vi "Measurement Logic.vi"() -> ()   [LabVIEW 2021, in "SourceMeasureDCVoltage.lvlib"]
uses:
  SourceMeasureDCVoltage.lvlib
  FAL/Functions/Measure_Voltage/Measure_Voltage.lvclass
  FAL/Functions/Source_Voltage/Source_Voltage.lvclass
  FAL/Instruments/Abstract_Instrument/Abstract_Instrument.lvclass
  Measurement Results.ctl
  FAL/Instruments/Abstract_Instrument/controls/Initialize_Info.ctl
  FAL/Instruments/Abstract_Instrument/Utility/Initialize N Pins.vi
  FAL/Functions/Measure_Voltage/Utility/Get 1 Object.vi
  FAL/Functions/Source_Voltage/Utility/Get 1 Object.vi
  <vilib>/Plug-In SDKs/Clients/Session Management V1/Session Reservation/Initialize and Close Session Behavior.ctl
  <vilib>/Plug-In SDKs/Clients/Session Management V1/Session Reservation/Session Reservation.lvclass
  3a97cad3-1174-4d4c-995c-4f8f4017f4b7.vi
  Measurement Configuration.ctl
  <vilib>/Plug-In SDKs/Measurements/Measure Call Context/Measure Call Context.lvclass
panel:
  out "measure call context out":refnum<class "Measure Call Context.lvclass">
  in  "measure call context in":refnum<class "Measure Call Context.lvclass">
  in  "measurement configuration":T1={"source_pin"="", "Voltage Level"=0.0, "Voltage Level Range"=0.0, "Current Limit"=0.0, "Current Limit Range"=0.0, "Source Delay (Sec)"=0.0, "measure_pin"="", "Resolution in Digits"=enum."5 1/2"}
  out "measurement results":T2 {"Measurement" format="%.6p"}
  out "error out":errorcluster
  in  "error in":errorcluster
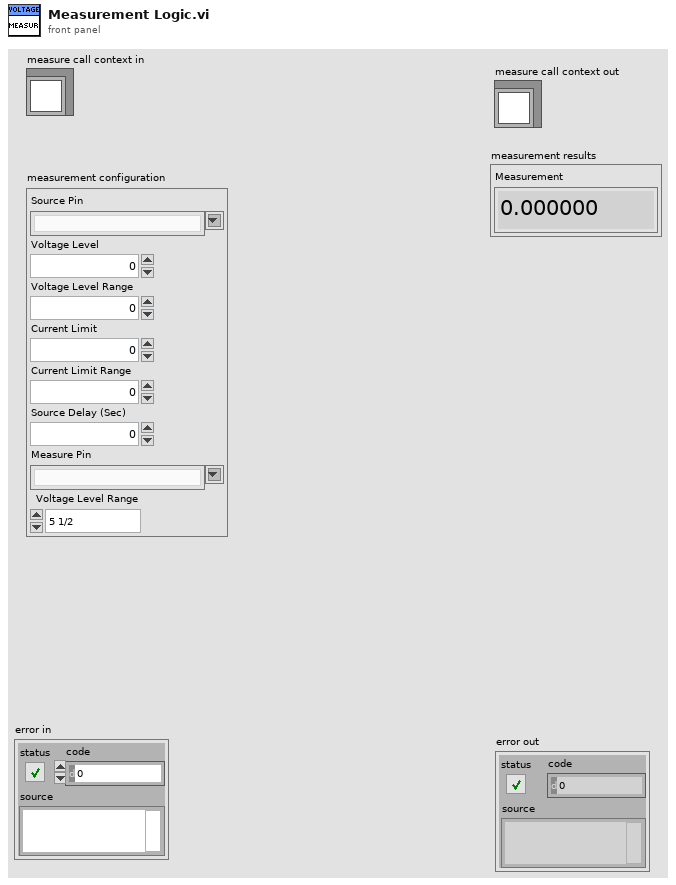
[diagram p1: front panel]
types:
  T1 = typedef "SourceMeasureDCVoltage.lvlib/Measurement Configuration.ctl" = cluster{"source_pin":string, "Voltage Level":dbl, "Voltage Level Range":dbl, "Current Limit":dbl, "Current Limit Range":dbl, "Source Delay (Sec)":dbl, "measure_pin":string, "Resolution in Digits":enum32{"3 1/2", "4 1/2", "5 1/2", "6 1/2", "7 1/2"}}
  T2 = typedef "SourceMeasureDCVoltage.lvlib/Measurement Results.ctl" = cluster{"Measurement":dbl}
  T3 = typedef "NI Session Management V1 Client.lvlib/Session Reservation.lvclass/Initialize and Close Session Behavior.ctl" = enum16{"Auto", "Initialize and Close", "Attach and Detach", "Initialize and Detach", "Attach and Close"}
  T4 = typedef "Abstract_Instrument.lvclass/Initialize_Info.ctl" = cluster{"initialize and close session behavior":T3, "reset":bool, "optional string":string}
  T5 = enum32{"3 1/2", "4 1/2", "5 1/2", "6 1/2", "7 1/2"}
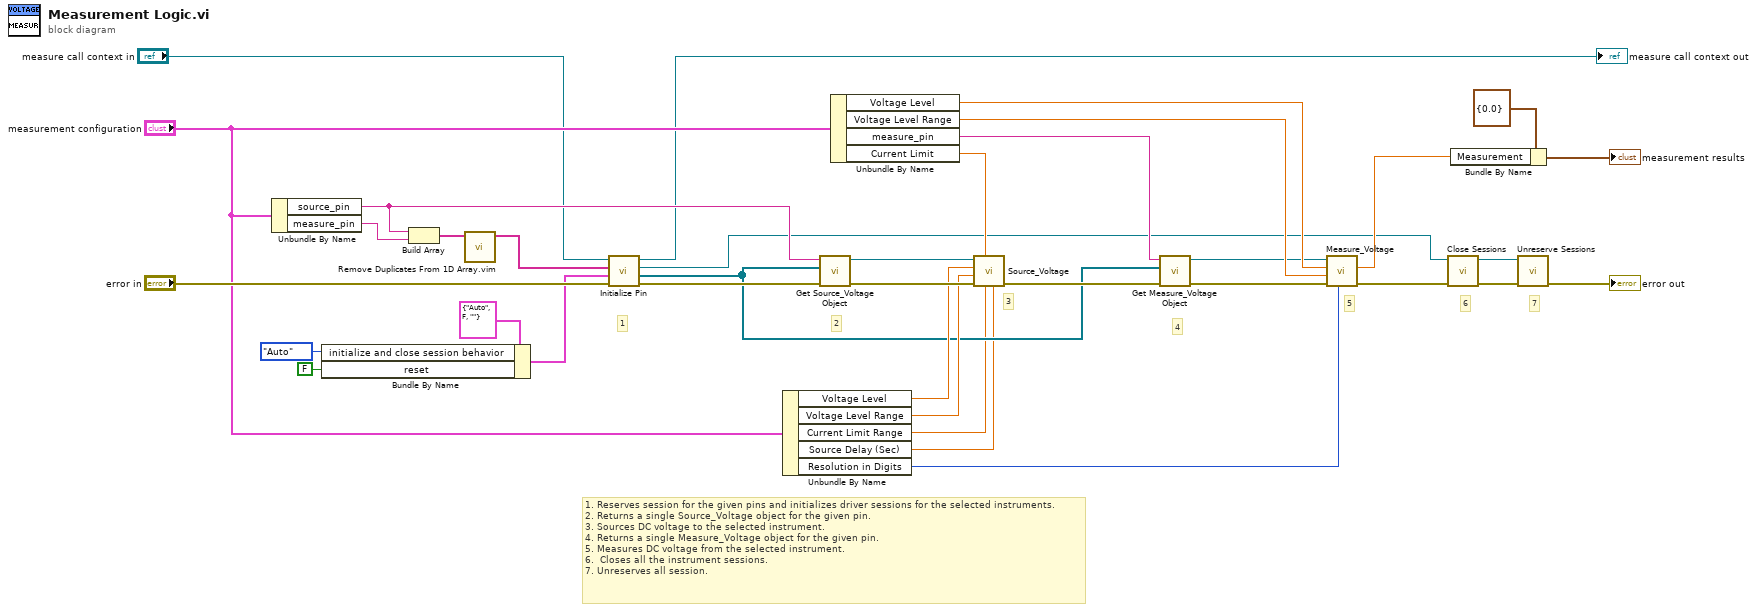
[diagram p0: block diagram]
diagram:
  # "1. Reserves session for the given pins and initializes driver sessions for the selected instruments.\n2. Returns a single Source_Voltage object for the given pin.\n3. Sources DC voltage to the selected instrument.\n4. Returns a single Measure_Voltage object for the given pin.\n5. Measures DC voltage from the selected instrument.\n6.  Closes all the instrument sessions.\n7. Unreserves all session."
  # "7"
  # "6"
  # "5"
  # "4"
  # "3"
  # "2"
  # "1"
  n1 = Unbundle By Name("measurement configuration") -> ("source_pin"=w24:string, "measure_pin"=w27:string)
  n2 = Bundle By Name(cluster=T4 {"initialize and close session behavior"=enum."Auto", "reset"=FALSE, "optional string"=""} ("Initialize_Info"), "initialize and close session behavior"=Initialize_and_Close_Session_Behavior."Auto", "reset"=FALSE) -> (w14:T4)
  n3 = Build Array(w24, w27) -> (w25:string[])
  n4 = call "Remove Duplicates From 1D Array.vim"("array"=w25) -> ("array with duplicates removed"=w6:string[])  [unwired: 10 in]
  n5 = call-poly "Initialize Pin.vi"("error in"="error in", "Initialize_Info"=w14, "pin or relay names"=w6, "measure call context in"="measure call context in") -> ("error out"=w26:errorcluster, "instrument object"=w21:refnum<class "Abstract_Instrument.lvclass">[], "session reservation out"=w2:refnum<class "Session Reservation.lvclass">, "measure call context out"=→"measure call context out":refnum<class "Measure Call Context.lvclass">)  [unwired: 4 in]
  n6 = Unbundle By Name("measurement configuration") -> ("Voltage Level"=w29:dbl, "Voltage Level Range"=w28:dbl, "Current Limit Range"=w11:dbl, "Source Delay (Sec)"=w10:dbl, "Resolution in Digits"=w5:T5)
  n7 = call-poly "Get Source_Voltage Object.vi"("error in"=w26, "instrument object"=w21, "pin_name"=w24) -> ("error out"=w31:errorcluster, "function object"=w23:refnum<class "Source_Voltage.lvclass">)  [unwired: 7 in]
  n8 = Unbundle By Name("measurement configuration") -> ("Voltage Level"=w4:dbl, "Voltage Level Range"=w3:dbl, "measure_pin"=w22:string, "Current Limit"=w12:dbl)
  n9 = call-dynamic "Source_Voltage.vi"("Source Delay (Sec)"=w10, "Current Limit Range"=w11, "Current Limit"=w12, "error in (no error)"=w31, "Voltage Level Range"=w28, "Voltage Level"=w29, "Source_Voltage in"=w23) -> ("error out"=w30:errorcluster)  [unwired: 3 in, 1 out]
  n10 = call-poly "Get Measure_Voltage Object.vi"("error in"=w30, "instrument object"=w21, "pin_name"=w22) -> ("error out"=w32:errorcluster, "function object"=w1:refnum<class "Measure_Voltage.lvclass">)  [unwired: 7 in]
  n11 = call-dynamic "Measure_Voltage.vi"("Resolution in Digits"=w5, "error in (no error)"=w32, "Range"=w3, "Level"=w4, "Measure_Voltage in"=w1) -> ("error out"=w34:errorcluster, "DC_Voltage"=w33:dbl)  [unwired: 3 in, 2 out]
  n12 = call <vilib>:"Close Sessions.vi"("error in"=w34, "session reservation in"=w2) -> ("error out"=w36:errorcluster, "session reservation out"=w35:refnum<class "Session Reservation.lvclass">)  [unwired: 8 in]
  n13 = Bundle By Name(cluster=T2 {"Measurement"=0.0} ("measurement results"), "Measurement"=w33) -> (→"measurement results":T2)
  n14 = call <vilib>:"Unreserve Sessions.vi"("error in"=w36, "session reservation in"=w35) -> ("error out"=→"error out":errorcluster)  [unwired: 9 in]
